vi "Main.vi"() -> ()   [LabVIEW 2018, in "Popup.lvlib"]
doc: "This template is based from the Queued Message Handler design pattern and the Queued Message Handler Project Template that ships with LabVIEW 2014.\n\nThe main difference is that the Queue is private to this module and communication between modules is done via Broadcast and Requests events.\n\nRequests events are wrapped via public API methods and are handled in the Event handler loop in this VI.\nAny module can register for Broadcast events sent by this module.\n\nThe Event Handling Loop generates messages based on user interface actions.\n\nThe Message Handling Loop processes messages generated by the Event Handling Loop, or by other messages. The messages are string values, so new messages can be added easily to the Message Cases case structure in the Message Handling Loop. Each message cluster can also provide an optional value for Message Data, which is a variant that can be converted to whatever message-specific data is required.\n_____\nBased on Delacor QMH Project Template 3.1.0.34."
uses:
  Popup.lvlib
  <vilib>/Delacor/Delacor QMH/Libraries/Cloneable Module Admin_class/Delacor_lib_QMH_Cloneable Module Admin.lvclass
  C:/Program Files (x86)/National Instruments/LabVIEW 2018/vi.lib/Delacor/Delacor QMH/Libraries/Module Admin_class/Delacor_lib_QMH_Module Admin.lvclass
  <vilib>/MGI/Panel Manager/Panel/Panel/Panel.lvclass
  <vilib>/Utility/miscctls.llb/LVPointTypeDef.ctl
  Module Data--cluster.ctl
  <vilib>/Delacor/Delacor QMH/Libraries/Message Queue_class/Delacor_lib_QMH_Message Queue.lvclass/Delacor_lib_QMH_Message Queue.ctl
  <vilib>/Delacor/Delacor QMH/Libraries/Cloneable Module Admin_class/Delacor_lib_QMH_Cloneable Module Admin.lvclass/Delacor_lib_QMH_Cloneable Module Admin.ctl
  Stop Argument--cluster.ctl
  <vilib>/Delacor/Delacor QMH/Libraries/Module Admin_class/Delacor_lib_QMH_Module Admin.lvclass/Delacor_lib_QMH_Module Admin.ctl
  modify panl  origin position Argument--cluster.ctl
  Modify window front Argument--cluster.ctl
  Modify Title name Argument--cluster.ctl
  <vilib>/Utility/miscctls.llb/LVRectTypeDef.ctl
  <vilib>/Delacor/Delacor QMH/Libraries/Message Queue_class/Delacor_lib_QMH_Enqueue Message (Single).vi
  <vilib>/Delacor/Delacor QMH/Libraries/Cloneable Module Admin_class/Delacor_lib_QMH_Get Module ID.vi
  <vilib>/Delacor/Delacor QMH/Libraries/Module Admin_class/Delacor_lib_QMH_Get External Launch.vi
  <vilib>/Utility/error.llb/Error Cluster From Error Code.vi
  <vilib>/ErrorRing/Error Ring.xnode
  <vilib>/Delacor/Delacor QMH/Libraries/Message Queue_class/Delacor_lib_QMH_Message Queue.lvclass
  Clone Registration/Clone Registration.lvlib
  <vilib>/MGI/Panel Manager/Panel/Panel Helper/Panel Helper.lvclass
panel:
  in  "显示字符串":string
  in  "Panel":refnum<class "Panel.lvclass">
  in  "Simulate MHL Error":bool
  in  "Simulate EHL Error":bool
  out "error out":errorcluster
  in  "Module Admin":refnum<class "Delacor_lib_QMH_Cloneable Module Admin.lvclass">
  out "Status":string
  # "一个模块涵盖所有弹窗\n所有对应操作全部通过命令下发"
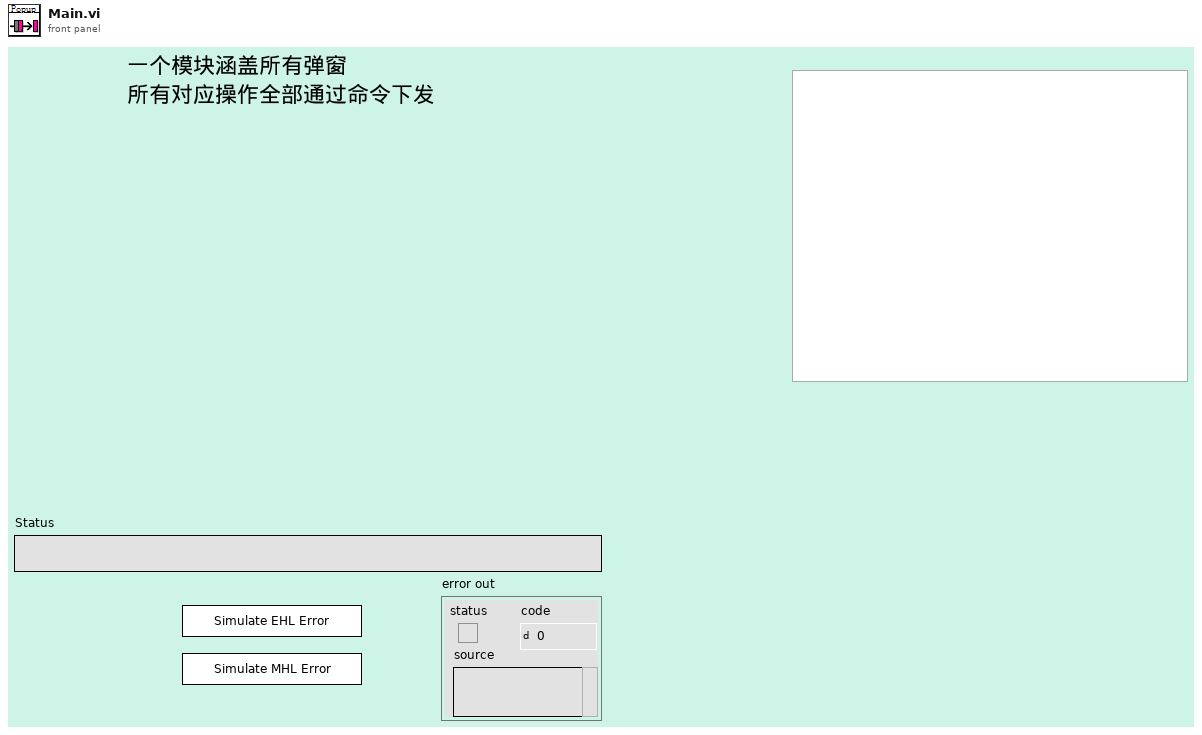
[diagram p1: front panel]
types:
  T1 = typedef "LVPointTypeDef.ctl" = cluster{"Horizontal":i16, "Vertical":i16}
  T2 = typedef "Popup.lvlib/Request Events--cluster.ctl" = cluster{"Stop Module":refnum<user-event>, "Show Panel":refnum<user-event>, "Hide Panel":refnum<user-event>, "Show Diagram":refnum<user-event>, "Get Module Execution Status":refnum<user-event>, "Change Panel":refnum<user-event>, "modify panl  origin position":refnum<user-event>, "Modify window front":refnum<user-event>, "Modify Title name":refnum<user-event>}
  T3 = typedef "Panel.lvlib/Panel Helper.lvclass/Panel Events.ctl" = cluster{"My Panel":refnum<user-event>, "Top Level Initialized":refnum<user-event>}
  T4 = typedef "Popup.lvlib/Module Data--cluster.ctl" = cluster{"Status":string, "本VI":refnum<vi>}
  T5 = typedef "Popup.lvlib/Stop Argument--cluster.ctl" = cluster{"Origin":string, "Module ID":i32, "Exit via Stop Module Req?":bool, "Wait for Module to stop?":bool}
  T6 = typedef "Popup.lvlib/modify panl  origin position Argument--cluster.ctl" = cluster{"Module ID":i32, "Origin":cluster{"Horizontal":i16, "Vertical":i16}}
  T7 = typedef "Popup.lvlib/Modify window front Argument--cluster.ctl" = cluster{"Module ID":i32, "Bottom":i16, "Right":i16, "Top":i16, "Left":i16}
  T8 = typedef "Popup.lvlib/Modify Title name Argument--cluster.ctl" = cluster{"Module ID":i32, "标题":string}
  T9 = enum32{"invalid lock state", "Not Locked", "Locked (No Password)", "Password-protected"}
  T10 = typedef "LVRectTypeDef.ctl" = cluster{"Left":i16, "Top":i16, "Right":i16, "Bottom":i16}
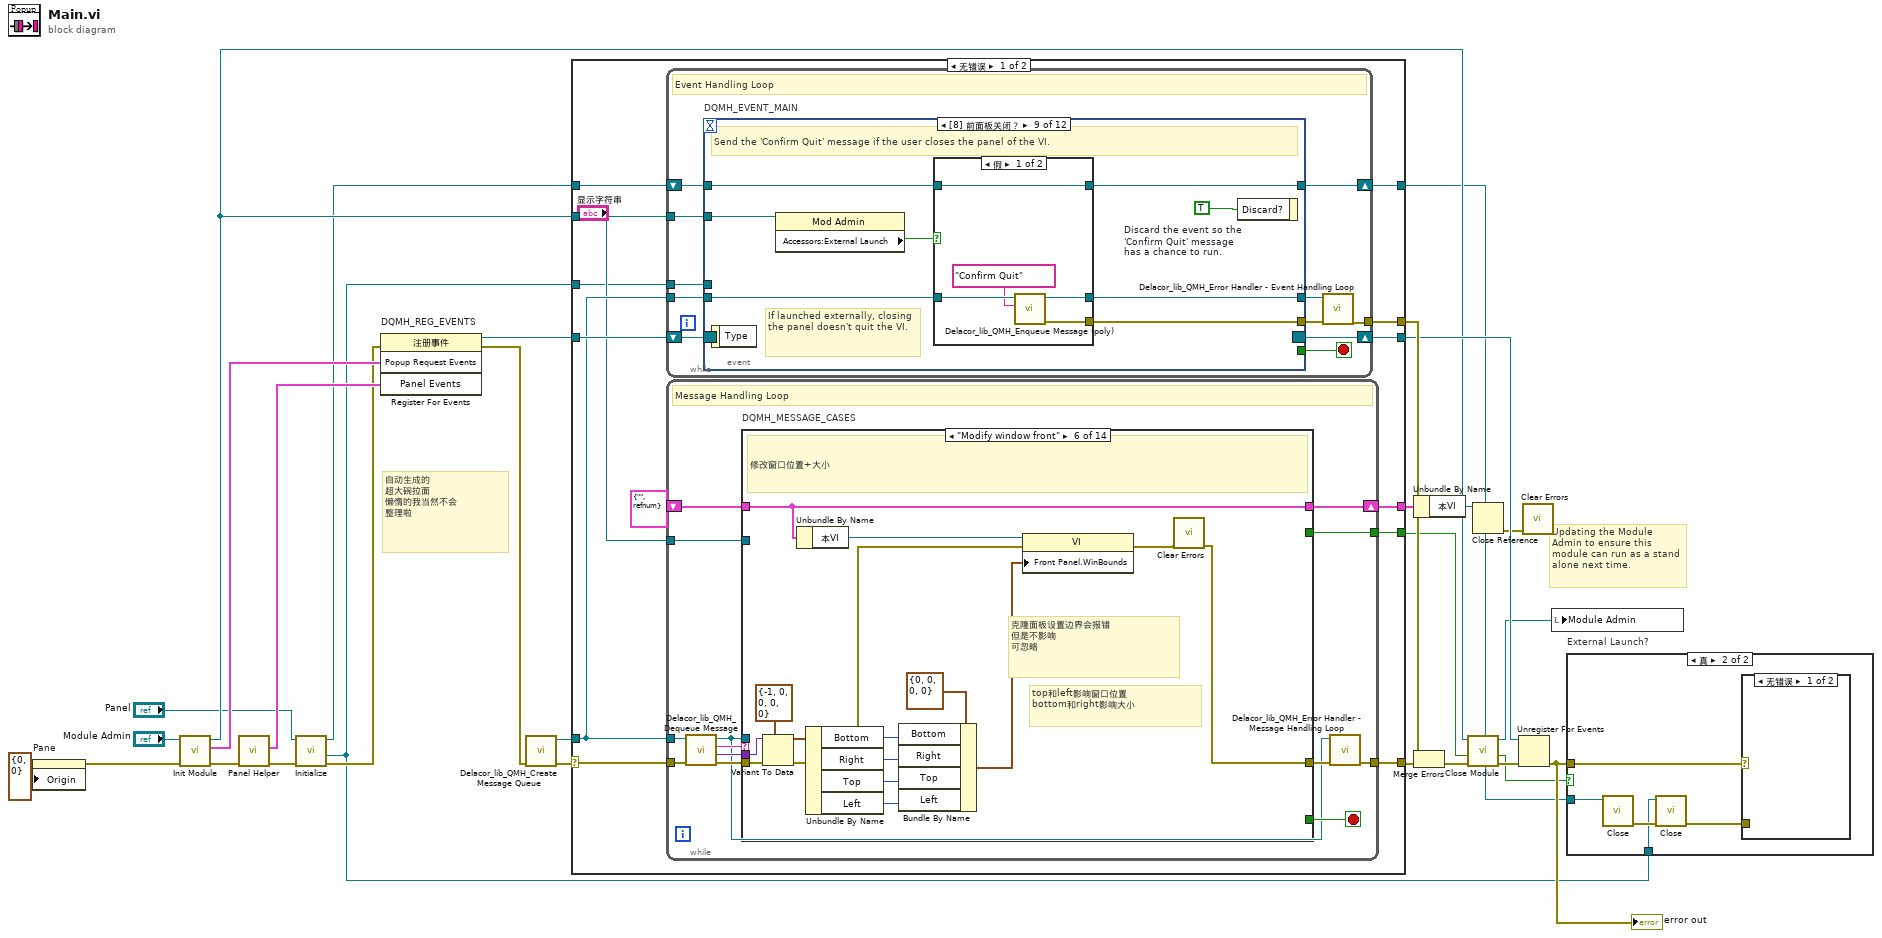
[diagram p0: block diagram]
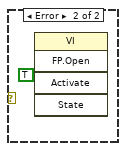
[diagram p3: hidden frame]
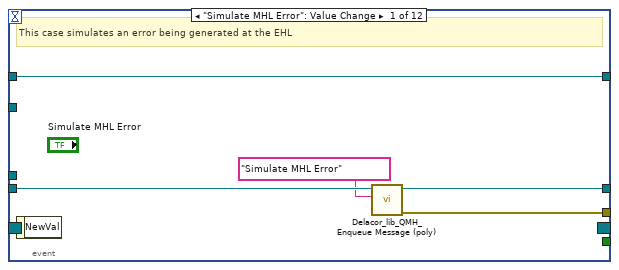
[diagram p4: hidden frame]
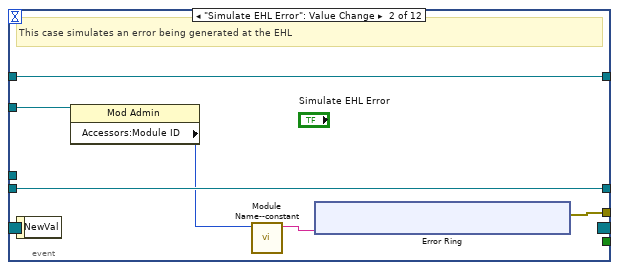
[diagram p5: hidden frame]
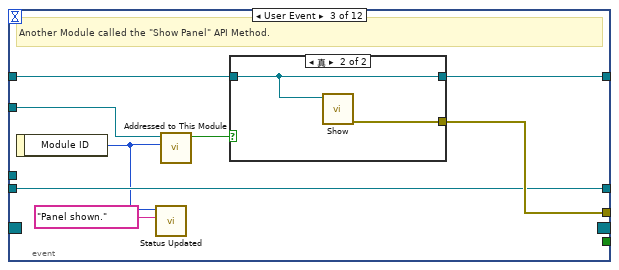
[diagram p6: hidden frame]
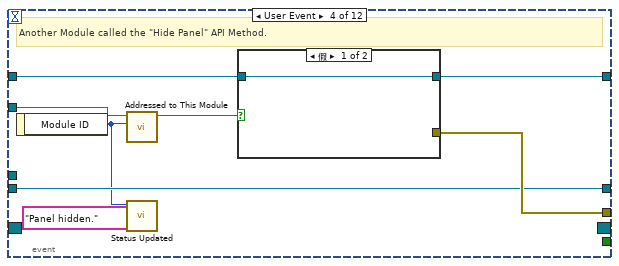
[diagram p8: hidden frame]
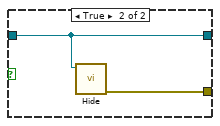
[diagram p9: hidden frame]
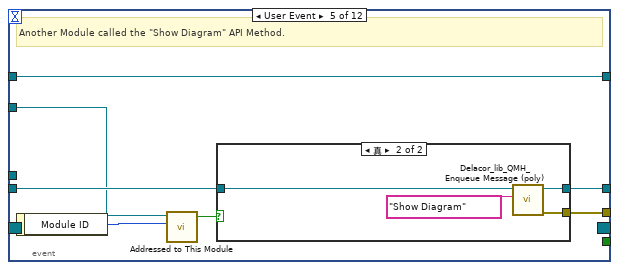
[diagram p10: hidden frame]
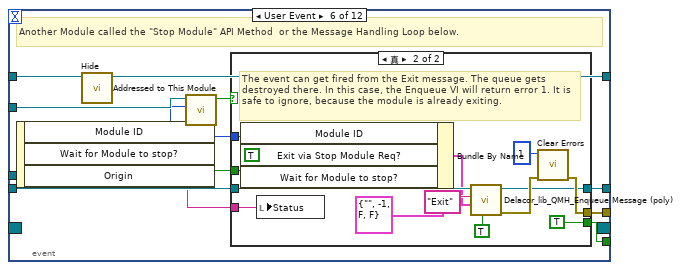
[diagram p12: hidden frame]
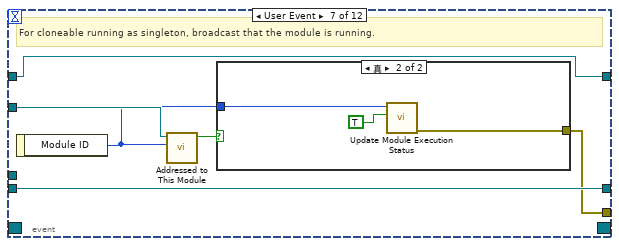
[diagram p14: hidden frame]
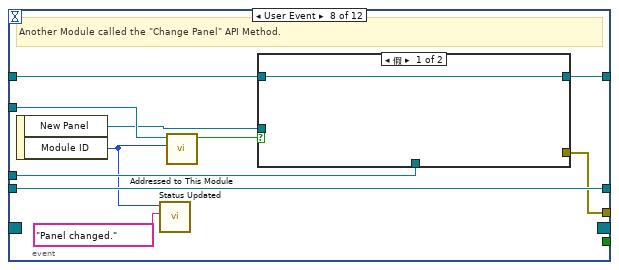
[diagram p16: hidden frame]
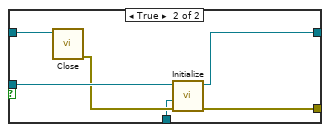
[diagram p17: hidden frame]
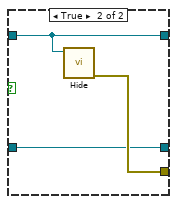
[diagram p18: hidden frame]
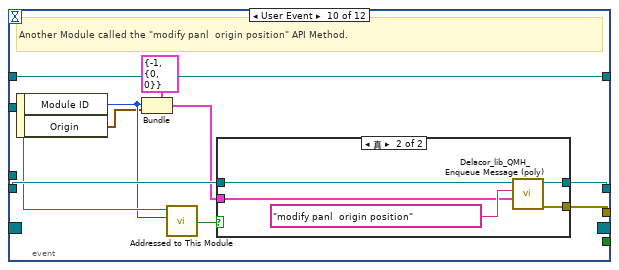
[diagram p19: hidden frame]
diagram:
  # "自动生成的\n超大碗拉面\n懒惰的我当然不会\n整理啦"
  # "Updating the Module Admin to ensure this module can run as a stand alone next time."
  n1 = property on="Pane" class="Pane"("Origin"=T1 {"Horizontal"=0, "Vertical"=0}) -> (error out=w4:errorcluster)  [unwired: 2 in, 1 out]
  n2 = call "Init Module.vi"("error in (no error)"=w4, "Cloneable Module Admin in"="Module Admin") -> ("error out"=w14:errorcluster, "Popup Request Events"=w24:T2, "Cloneable Module Admin out"=w20:refnum<class "Delacor_lib_QMH_Cloneable Module Admin.lvclass">)  [unwired: 7 in]
  n3 = call <vilib>:"Panel Helper.vi"("Error In"=w14) -> ("Error Out"=w10:errorcluster, "Panel Events"=w13:T3)  [unwired: 8 in, 1 out]
  n4 = call <vilib>:"Initialize.vi"("error in (no error)"=w10, "Panel In"="Panel") -> ("error out"=w9:errorcluster, "My Helper out"=w6:refnum<class "Panel Helper.lvclass">, "Panel Out"=w7:refnum<class "Panel.lvclass">)  [unwired: 7 in]
  n5 = register-events "DQMH_REG_EVENTS"(error in=w9, w24, w13) -> (reference out=w25:refnum<event-registration>, error out=w11:errorcluster)  [unwired: 1 in]
  n6 = call <vilib>:"Delacor_lib_QMH_Create Message Queue.vi"("error in"=w11) -> ("error out"=w15:errorcluster, "Message Queue"=w23:refnum<class "Delacor_lib_QMH_Message Queue.lvclass">)  [unwired: 9 in]
  n7 = case shown="无错误" w15 {
    selector: w15 -> [w36 w403]
    tunnel: [w42 w403] -> w27
    tunnel: [w41 w404] -> w26
    tunnel: w25 -> [w39 w404]
    tunnel: w23 -> [w38 _]
    tunnel: [w37 _] -> w28
    tunnel: w20 -> [w35 w399]
    tunnel: [w34 _] -> w18
    tunnel: w6 -> [w31 _]
    tunnel: w7 -> [w33 w396]
    tunnel: [w32 w396] -> w12
    tunnel: [w30 _] -> w3
    frame No Error {
      n8 = while {
        tunnel: w38 -> [w53]
        shift-right: [w51] -> w41
        shift-left: w39 -> [w52]
        tunnel: [w47] -> w37
        tunnel: w35 -> [w46]
        shift-right: [w44] -> w32
        shift-left: w33 -> [w45]
        tunnel: w31 -> [w43]
        stop <- w49 stop-if-true
        # "Event Handling Loop"
        n9 = event "DQMH_EVENT_MAIN" shown="[8] 前面板关闭？" {
          selector: w52 -> [_ _ _ _ _ _ _ _ _ _ _ _]
          dyn-events: [_ _ _ _ _ _ _ _ _ _ _ _] -> w51
          timeout: _ -> [_ _ _ _ _ _ _ _ _ _ _ _]
          tunnel: [_ _ _ _ _ w110 _ _ _ _ _ _] -> w49
          tunnel: w53 -> [w58 w64 w74 w85 w100 w113 w134 w146 w158 w181 w200 w216]
          tunnel: [w56 w63 w79 w90 w96 w115 w133 w144 w157 w173 w189 w208] -> w50
          tunnel: [w57 w64 w74 w85 w99 w114 w134 w146 w159 w180 w199 w215] -> w48
          tunnel: w46 -> [_ w62 w77 w88 w97 w112 w135 w149 w163 w178 w197 w213]
          tunnel: w45 -> [w54 w59 w76 w86 w94 w106 w131 w148 w162 w182 w201 w217]
          tunnel: [w54 w59 w75 w87 w94 w106 w131 w147 w161 w182 w201 w217] -> w44
          tunnel: w43 -> [_ _ _ _ _ _ _ w143 _ _ _ _]
          event "Simulate MHL Error": Value Change {
            # "This case simulates an error being generated at the EHL"
            n10 = event-data() -> ()  [unwired: 1 in, 1 out]
            n11 = call-poly <vilib>:"Delacor_lib_QMH_Enqueue Message (poly).vi"("Message"="Simulate MHL Error", "Message Queue in"=w58) -> ("error out"=w56:errorcluster, "Message Queue out"=w57:refnum<class "Delacor_lib_QMH_Message Queue.lvclass">)  [unwired: 8 in]
          }
          event "Simulate EHL Error": Value Change {
            # "This case simulates an error being generated at the EHL"
            n12 = event-data() -> ()  [unwired: 1 in, 1 out]
            n13 = property class="Mod Admin"(reference=w62) -> ("Accessors:Module ID"=w61:i32)  [unwired: 1 in, 2 out]
            n14 = call "Module Name--constant.vi"("Module ID"=w61) -> ("Module Name"=w60:string)  [unwired: 10 in]
            n15 = xnode "Error Ring"("参数 0"=w60) -> ("错误输出"=w63:errorcluster)
          }
          event User Event {
            # "Another Module called the \"Show Panel\" API Method."
            n16 = event-data() -> ("Module ID"=w72:i32)  [unwired: 1 in]
            n17 = call "Status Updated.vi"("Status"="Panel shown." ("format string"), "Module ID"=w72) -> ()  [unwired: 9 in, 1 out]
            n18 = call "Addressed to This Module.vi"("Module ID from Argument"=w72, "Module Admin"=w77) -> ("Addressed to this instance?"=w78:bool)  [unwired: 8 in, 1 out]
            n19 = case shown="真" w78 {
              tunnel: [_ w81] -> w79
              tunnel: w76 -> [w80 w82]
              tunnel: [w80 w82] -> w75
              frame False {
              }
              frame True {
                n20 = call <vilib>:"Show.vi"("Panel in"=w82) -> ("Error Out"=w81:errorcluster)  [unwired: 10 in]
              }
            }
          }
          event User Event {
            # "Another Module called the \"Hide Panel\" API Method."
            n21 = event-data() -> ("Module ID"=w83:i32)  [unwired: 1 in]
            n22 = call "Addressed to This Module.vi"("Module ID from Argument"=w83, "Module Admin"=w88) -> ("Addressed to this instance?"=w89:bool)  [unwired: 8 in, 1 out]
            n23 = call "Status Updated.vi"("Status"="Panel hidden." ("format string"), "Module ID"=w83) -> ()  [unwired: 9 in, 1 out]
            n24 = case shown="假" w89 {
              tunnel: [_ w92] -> w90
              tunnel: [w91 w93] -> w87
              tunnel: w86 -> [w91 w93]
              frame False {
              }
              frame True {
                n25 = call <vilib>:"Hide.vi"("Panel In"=w93) -> ("Error Out"=w92:errorcluster)  [unwired: 10 in]
              }
            }
          }
          event User Event {
            # "Another Module called the \"Show Diagram\" API Method."
            n26 = event-data() -> ("Module ID"=w95:i32)  [unwired: 1 in]
            n27 = call "Addressed to This Module.vi"("Module ID from Argument"=w95, "Module Admin"=w97) -> ("Addressed to this instance?"=w98:bool)  [unwired: 8 in, 1 out]
            n28 = case shown="真" w98 {
              tunnel: w100 -> [w101 w105]
              tunnel: [w101 w104] -> w99
              tunnel: [_ w102] -> w96
              frame False {
              }
              frame True {
                n29 = call-poly <vilib>:"Delacor_lib_QMH_Enqueue Message (poly).vi"("Message"="Show Diagram", "Message Queue in"=w105) -> ("error out"=w102:errorcluster, "Message Queue out"=w104:refnum<class "Delacor_lib_QMH_Message Queue.lvclass">)  [unwired: 8 in]
              }
            }
          }
          event User Event {
            # "Another Module called the \"Stop Module\" API Method  or the Message Handling Loop below."
            n30 = event-data() -> ("Module ID"=w108:i32, "Wait for Module to stop?"=w109:bool, "Origin"=w107:string)  [unwired: 1 in]
            n31 = call <vilib>:"Hide.vi"("Panel In"=w106) -> ()  [unwired: 10 in, 1 out]
            n32 = call "Addressed to This Module.vi"("Module ID from Argument"=w108, "Module Admin"=w112) -> ("Addressed to this instance?"=w111:bool)  [unwired: 8 in, 1 out]
            n33 = case shown="真" w111 {
              tunnel: [_ w126] -> w115
              tunnel: [w116 w125] -> w114
              tunnel: w113 -> [w116 w124]
              tunnel: [_ TRUE] -> w110
              tunnel: w109 -> [_ w119]
              tunnel: w108 -> [_ w121]
              tunnel: w107 -> [_ w117]
              frame False {
              }
              frame True {
                # "The event can get fired from the Exit message. The queue gets destroyed there. In this case, the Enqueue VI will return error 1. It is safe to ignore, because the module is already exiting."
                n34 = Bundle By Name(cluster=T5 {"Origin"="", "Module ID"=-1, "Exit via Stop Module Req?"=FALSE, "Wait for Module to stop?"=FALSE} ("Stop Argument"), "Module ID"=w121, "Exit via Stop Module Req?"=TRUE, "Wait for Module to stop?"=w119) -> (w118:T5)
                n35 = local write "Status"(w117) -> ()
                n36 = call-poly <vilib>:"Delacor_lib_QMH_Enqueue Message (poly).vi"("Priority Message? (F)"=TRUE, "Message Data"=w118, "Message"="Exit", "Message Queue in"=w124) -> ("error out"=w129:errorcluster, "Message Queue out"=w125:refnum<class "Delacor_lib_QMH_Message Queue.lvclass">)  [unwired: 6 in]
                n37 = call <vilib>:"Clear Errors.vi"("error in (no error)"=w129, "specific error code to clear (0: all)"=1) -> ("error out"=w126:errorcluster)  [unwired: 4 in, 1 out]
              }
            }
          }
          event User Event {
            # "For cloneable running as singleton, broadcast that the module is running."
            n38 = event-data() -> ("Module ID"=w132:i32)  [unwired: 1 in]
            n39 = call "Addressed to This Module.vi"("Module ID from Argument"=w132, "Module Admin"=w135) -> ("Addressed to this instance?"=w136:bool)  [unwired: 8 in, 1 out]
            n40 = case shown="真" w136 {
              tunnel: [_ w139] -> w133
              tunnel: w132 -> [_ w138]
              frame False {
              }
              frame True {
                n41 = call "Update Module Execution Status.vi"("Running?"=TRUE, "Module ID"=w138) -> ("error out"=w139:errorcluster)  [unwired: 9 in]
              }
            }
          }
          event User Event {
            # "Another Module called the \"Change Panel\" API Method."
            n42 = event-data() -> ("New Panel"=w145:refnum<class "Panel.lvclass">, "Module ID"=w141:i32)  [unwired: 1 in]
            n43 = call "Status Updated.vi"("Status"="Panel changed.", "Module ID"=w141) -> ()  [unwired: 9 in, 1 out]
            n44 = call "Addressed to This Module.vi"("Module ID from Argument"=w141, "Module Admin"=w149) -> ("Addressed to this instance?"=w140:bool)  [unwired: 8 in, 1 out]
            n45 = case shown="假" w140 {
              tunnel: w148 -> [w150 w156]
              tunnel: [w150 w154] -> w147
              tunnel: w145 -> [_ w155]
              tunnel: [_ w152] -> w144
              tunnel: w143 -> [_ w151]
              frame False {
              }
              frame True {
                n46 = call-dynamic <vilib>:"Close.vi"("Panel In"=w156) -> ("Error Out"=w153:errorcluster)  [unwired: 10 in]
                n47 = call <vilib>:"Initialize.vi"("error in (no error)"=w153, "My Helper in"=w151, "Panel In"=w155) -> ("error out"=w152:errorcluster, "Panel Out"=w154:refnum<class "Panel.lvclass">)  [unwired: 6 in, 1 out]
              }
            }
          }
          event Panel Close? {
            w164 = TRUE  # Discard the event so the 'Confirm Quit' message has a chance to run.
            # "If launched externally, closing the panel doesn't quit the VI."
            # "Send the 'Confirm Quit' message if the user closes the panel of the VI."
            n48 = event-data() -> ()  [unwired: 1 in, 1 out]
            n49 = property class="Mod Admin"(reference=w163) -> ("Accessors:External Launch"=w160:bool)  [unwired: 1 in, 2 out]
            n50 = case "条件结构" shown="假" w160 {
              tunnel: w162 -> [w167 w172]
              tunnel: [w167 w172] -> w161
              tunnel: [w166 w171] -> w157
              tunnel: [w168 w170] -> w159
              tunnel: w158 -> [w169 w170]
              frame False {
                n51 = call-poly <vilib>:"Delacor_lib_QMH_Enqueue Message (poly).vi"("Message"="Confirm Quit", "Message Queue in"=w169) -> ("error out"=w166:errorcluster, "Message Queue out"=w168:refnum<class "Delacor_lib_QMH_Message Queue.lvclass">)  [unwired: 8 in]
              }
              frame True {
                n52 = call <vilib>:"Hide.vi"("Panel In"=w172) -> ("Error Out"=w171:errorcluster)  [unwired: 10 in]
              }
            }
            n53 = event-data("Discard?"=w164) -> ()  [unwired: 1 in, 1 out]
          }
          event User Event {
            # "Another Module called the \"modify panl  origin position\" API Method."
            n54 = event-data() -> ("Module ID"=w175:i32, "Origin"=w174:cluster{"Horizontal":i16, "Vertical":i16})  [unwired: 1 in]
            n55 = Bundle(cluster=T6 {"Module ID"=-1, "Origin"={"Horizontal"=0, "Vertical"=0}} ("modify panl  origin position Argument"), "Module ID"=w175, "Origin"=w174) -> (w176:T6)
            n56 = call "Addressed to This Module.vi"("Module ID from Argument"=w175, "Module Admin"=w178) -> ("Addressed to this instance?"=w179:bool)  [unwired: 8 in, 1 out]
            n57 = case "条件结构" shown="真" w179 {
              tunnel: w181 -> [w183 w188]
              tunnel: [w183 w187] -> w180
              tunnel: w176 -> [_ w185]
              tunnel: [_ w184] -> w173
              frame False {
              }
              frame True {
                n58 = call-poly <vilib>:"Delacor_lib_QMH_Enqueue Message (poly).vi"("Message Data"=w185, "Message"="modify panl  origin position", "Message Queue in"=w188) -> ("error out"=w184:errorcluster, "Message Queue out"=w187:refnum<class "Delacor_lib_QMH_Message Queue.lvclass">)  [unwired: 7 in]
              }
            }
          }
          event User Event {
            # "Another Module called the \"Modify window front\" API Method."
            n59 = event-data() -> ("Module ID"=w194:i32, "Bottom"=w193:i16, "Right"=w192:i16, "Top"=w191:i16, "Left"=w190:i16)  [unwired: 1 in]
            n60 = Bundle(cluster=T7 {"Module ID"=-1, "Bottom"=0, "Right"=0, "Top"=0, "Left"=0} ("Modify window front Argument"), "Module ID"=w194, "Bottom"=w193, "Right"=w192, "Top"=w191, "Left"=w190) -> (w195:T7)
            n61 = call "Addressed to This Module.vi"("Module ID from Argument"=w194, "Module Admin"=w197) -> ("Addressed to this instance?"=w198:bool)  [unwired: 8 in, 1 out]
            n62 = case "条件结构" shown="真" w198 {
              tunnel: w200 -> [w202 w207]
              tunnel: [w202 w206] -> w199
              tunnel: w195 -> [_ w204]
              tunnel: [_ w203] -> w189
              frame False {
              }
              frame True {
                n63 = call-poly <vilib>:"Delacor_lib_QMH_Enqueue Message (poly).vi"("Message Data"=w204, "Message"="Modify window front", "Message Queue in"=w207) -> ("error out"=w203:errorcluster, "Message Queue out"=w206:refnum<class "Delacor_lib_QMH_Message Queue.lvclass">)  [unwired: 7 in]
              }
            }
          }
          event User Event {
            # "Another Module called the \"Modify Title name\" API Method."
            n64 = event-data() -> ("Module ID"=w210:i32, "标题"=w209:string)  [unwired: 1 in]
            n65 = Bundle(cluster=T8 {"Module ID"=-1, "标题"=""} ("Modify Title name Argument"), "Module ID"=w210, "标题"=w209) -> (w211:T8)
            n66 = call "Addressed to This Module.vi"("Module ID from Argument"=w210, "Module Admin"=w213) -> ("Addressed to this instance?"=w214:bool)  [unwired: 8 in, 1 out]
            n67 = case "条件结构" shown="真" w214 {
              tunnel: w216 -> [w218 w223]
              tunnel: [w218 w222] -> w215
              tunnel: w211 -> [_ w220]
              tunnel: [_ w219] -> w208
              frame False {
              }
              frame True {
                n68 = call-poly <vilib>:"Delacor_lib_QMH_Enqueue Message (poly).vi"("Message Data"=w220, "Message"="Modify Title name", "Message Queue in"=w223) -> ("error out"=w219:errorcluster, "Message Queue out"=w222:refnum<class "Delacor_lib_QMH_Message Queue.lvclass">)  [unwired: 7 in]
              }
            }
          }
        }
        n69 = call-dynamic "Delacor_lib_QMH_Error Handler - Event Handling Loop.vi"("error in"=w50, "Message Queue in"=w48) -> ("dup error in"=w47:errorcluster)  [unwired: 8 in, 1 out]
      }
      n70 = while {
        tunnel: w38 -> [w228]
        shift-right: [w234] -> w30
        shift-left: T4 {"Status"="", "本VI"=refnum} ("Data Cluster") -> [w235]
        tunnel: w36 -> [w232]
        tunnel: [w226] -> w42
        tunnel: w35 -> [w225]
        tunnel: [w224] -> w34
        stop <- w233 stop-if-true
        # "Message Handling Loop"
        n71 = call-dynamic "Delacor_lib_QMH_Dequeue Message.vi"("error in"=w232, "Message Queue in"=w228) -> ("error out"=w231:errorcluster, "Message Data"=w229:variant, "Message"=w230:string, "Message Queue out"=w227:refnum<class "Delacor_lib_QMH_Message Queue.lvclass">)  [unwired: 6 in]
        n72 = case "DQMH_MESSAGE_CASES" shown="\"Modify window front\"" w230 {
          selector: w230 -> [_ _ _ _ _ _ _ _ _ _ _ _ _ w385]
          tunnel: w227 -> [_ _ _ _ _ _ _ _ _ w330 _ w363 w379 _]
          tunnel: w231 -> [w248 w256 w261 w282 w298 w313 w322 w325 w328 w339 w352 w362 w381 _]
          tunnel: [w243 w257 w260 w280 w292 w300 w314 w323 w326 w329 w350 w361 w375 w386] -> w236
          tunnel: w235 -> [w247 w258 w262 w281 w297 w310 w318 w324 w327 w338 w351 w366 w378 w387]
          tunnel: [w246 w258 w262 w281 w297 w310 w318 w324 w327 w338 w351 w366 w378 w387] -> w234
          tunnel: [_ _ _ _ _ _ _ _ _ _ _ _ w377 _] -> w233
          tunnel: w229 -> [_ w255 _ _ w296 w312 w321 _ _ w337 _ _ w371 _]
          tunnel: w225 -> [w241 w250 w259 _ _ _ _ _ _ w334 w347 _ w367 w383]
          tunnel: [_ _ _ _ _ _ _ _ _ _ _ _ w369 _] -> w224
          frame "Initialize" {
            w245 = "Initial Message" ("Initial Message")
            # "#CodeNeeded - Initialize the appearance of the front panel."
            # "#CodeNeeded - Initialize your state data here."
            # "Initialize - Any operation that needs to be done before the module can receive messages. Synchronize Caller Events.vi will inform Start Module.vi that the module has launched and is ready to receive messages. Module Did Init.vi will broadcast that the module initialized."
            n73 = call "Synchronize Caller Events.vi"("error in (no error)"=w248, "Module Admin"=w241) -> ("error out"=w239:errorcluster, "Module Admin out"=w240:refnum<class "Delacor_lib_QMH_Cloneable Module Admin.lvclass">)  [unwired: 8 in]
            n74 = property class="Mod Admin"(reference=w240) -> ("Accessors:Module ID"=w242:i32)  [unwired: 1 in, 2 out]
            n75 = call "Module Name--constant.vi"("Module ID"=w242) -> ("Module Name"=w238:string)  [unwired: 10 in]
            n76 = control-ref of="本VI"() -> (w237:refnum<vi>)
            n77 = Bundle By Name(cluster=w247, "Status"=w245, "本VI"=w237) -> (w246:T4)
            n78 = local write "Status"(w245) -> ()
            n79 = call "Module Did Init.vi"("error in (no error)"=w239, "Initialized?"=TRUE, "Origin"=w238, "Module ID"=w242) -> ("error out"=w243:errorcluster)  [unwired: 7 in]
          }
          frame "Update Display" {
            # "Broadcast updated status to any VI registered to listen to this module's broadcast events."
            # "Convert the message data to a string to display in the Status indicator."
            # "#CodeRecommended - If you wish to decouple the Message Handling Loop from your user interface, consider creating User Events (like the \"Stop\" event in this VI) to message the Event Handling Loop whenever the user interface needs updating."
            # "Update Display - Update user interface here."
            n80 = Variant To Data(error in=w256, type="" ("空字符串常量"), Variant=w255) -> (data=w253:string, error out=w252:errorcluster)
            "Status" <- w253
            n81 = property class="Mod Admin"(reference=w250) -> ("Accessors:Module ID"=w249:i32)  [unwired: 1 in, 2 out]
            n82 = call "Status Updated.vi"("error in (no error)"=w252, "Status"=w253, "Module ID"=w249) -> ("error out"=w251:errorcluster)  [unwired: 8 in]
            n83 = Merge Errors(w251) -> (w257:errorcluster)
          }
          frame "Show Diagram" {
            # "Show Diagram - Show the block diagram of this VI. Used as a debugging tool. There is a button in the module tester that fires the Show Diagram request, which runs this message. Note that the diagram will not be displayed if it is password-protected and the password is not in the cache."
            n84 = disable-structure shown="RUN_TIME_ENGINE==False" {
              disable-tunnel: [w271 w279] -> w260
              disable-tunnel: w261 -> [w270 w279]
              disable-tunnel: w259 -> [w263 _]
              frame condition #0 (active) {
                # "functionality not available in exe"
                n85 = invoke class="VI" method="Lock State.Get"(error in=w270) -> (error out=w269:errorcluster, "Get Lock State"=w268:T9, "pwd in cache"=w265:bool)  [unwired: 3 in, 1 out]
                n86 = Equal?(x=T9."Password-protected", y=w268) -> (x = y?=w266:bool)
                n87 = Compound Arithmetic op=AND(w266, invert w265) -> (w264:bool)
                n88 = case shown="假" w264 {
                  tunnel: [w276 w278] -> w271
                  tunnel: w269 -> [w275 w278]
                  tunnel: w263 -> [w272 _]
                  frame False {
                    n89 = property class="Mod Admin"(reference=w272) -> ("Accessors:Module ID"=w273:i32)  [unwired: 1 in, 2 out]
                    n90 = property class="VI"(error in=w275, "BDWin.Open"=TRUE ("Block Diagram Window:Open")) -> (error out=w276:errorcluster)  [unwired: 1 in, 1 out]
                    n91 = call "Status Updated.vi"("Status"="Block Diagram shown." ("format string"), "Module ID"=w273) -> ()  [unwired: 9 in, 1 out]
                  }
                  frame True {
                    # "Password-protected VI, and the password is not in the cache. Do not show the diagram."
                  }
                }
              }
              frame condition #1 {
              }
            }
          }
          frame "--- Module Specific ---" {
            # "Separator -- The following cases handle messages specific to this Module."
            n92 = Merge Errors(w282) -> (w280:errorcluster)
          }
          frame "modify panl  origin position" {
            # "修改前面板原点位位置以达到换一块新的地方出来"
            n93 = Variant To Data(error in=w298, type=T6 {"Module ID"=-1, "Origin"={"Horizontal"=0, "Vertical"=0}} ("modify panl  origin position Argument"), Variant=w296) -> (data=w294:T6, error out=w293:errorcluster)
            n94 = Unbundle By Name(w294) -> ("Module ID"=w289:i32, "Origin"=w291:cluster{"Horizontal":i16, "Vertical":i16})
            n95 = Unbundle By Name(w291) -> ("Horizontal"=w287:i16, "Vertical"=w283:i16)
            n96 = property on="Pane" class="Pane"(error in=w293, "Origin"=w291) -> (error out=w288:errorcluster)  [unwired: 1 in, 1 out]
            n97 = Format Into String(format string="（%d，%d）" ("格式字符串"), initial string="modified origin position" ("输入字符串"), error in=w288, w287, w283) -> (resulting string=w286:string, error out=w285:errorcluster)
            n98 = call "Status Updated.vi"("error in (no error)"=w285, "Status"=w286, "Module ID"=w289) -> ("error out"=w292:errorcluster)  [unwired: 8 in]
          }
          frame "Modify window front" {
            # "top和left影响窗口位置\nbottom和right影响大小"
            # "克隆面板设置边界会报错\n但是不影响\n可忽略"
            # "修改窗口位置+大小"
            n99 = Variant To Data(error in=w313, type=T7 {"Module ID"=-1, "Bottom"=0, "Right"=0, "Top"=0, "Left"=0} ("Modify window front Argument"), Variant=w312) -> (data=w306:T7, error out=w308:errorcluster)
            n100 = Unbundle By Name(w310) -> ("本VI"=w309:refnum<vi>)
            n101 = Unbundle By Name(w306) -> ("Bottom"=w305:i16, "Right"=w304:i16, "Top"=w303:i16, "Left"=w302:i16)
            n102 = Bundle By Name(cluster=T10 {"Left"=0, "Top"=0, "Right"=0, "Bottom"=0} ("前面板窗口:窗口边界"), "Bottom"=w305, "Right"=w304, "Top"=w303, "Left"=w302) -> (w299:T10)
            n103 = property class="VI"(reference=w309, error in=w308, "Front Panel.WinBounds"=w299) -> (error out=w301:errorcluster)  [unwired: 1 out]
            n104 = call <vilib>:"Clear Errors.vi"("error in (no error)"=w301) -> ("error out"=w300:errorcluster)  [unwired: 5 in, 1 out]
          }
          frame "Modify Title name" {
            # "修改标题栏"
            n105 = Variant To Data(error in=w322, type=T8 {"Module ID"=-1, "标题"=""} ("Modify Title name Argument"), Variant=w321) -> (data=w319:T8, error out=w315:errorcluster)
            n106 = Unbundle By Name(w319) -> ("标题"=w316:string)
            n107 = Unbundle By Name(w318) -> ("本VI"=w317:refnum<vi>)
            n108 = property class="VI"(reference=w317, error in=w315, "Front Panel.Title"=w316) -> (error out=w314:errorcluster)  [unwired: 1 out]
          }
          frame "---Copy This Frame---" {
            # "Duplicate this frame when creating new messages.  Change this comment in the duplicated frame to describe this message."
            n109 = Merge Errors(w325) -> (w323:errorcluster)
          }
          frame "--- Exit and Error Handling---" {
            # "Separator - the following cases handle errors and exit messages."
            n110 = Merge Errors(w328) -> (w326:errorcluster)
          }
          frame "Error" {
            # "#CodeRecommended - If you ever change the name of this \"Error\" message, you'll need to update the name in the Check Loop Error.vi as well."
            # "#CodeRecommended - If the module is running in standalone mode (External Launch = FALSE), this code will pop up an error dialog and call the 'Exit' message if an error occurs. Add more fine-grained error handling here."
            # "Error - Check the error message data and respond accordingly. This message is sent by the \"Error Handler\" VIs at the end of each loop in this application."
            n111 = property class="Mod Admin"(reference=w334) -> ("Accessors:External Launch"=w331:bool, "Accessors:Module ID"=w333:i32)  [unwired: 1 in, 2 out]
            n112 = Variant To Data(error in=w339, type=errorcluster {"status"=FALSE, "code"=0, "source"=""} ("error constant"), Variant=w337) -> (data=w340:errorcluster, error out=w335:errorcluster)
            n113 = call "Error Reported.vi"("Error"=w340, "Module ID"=w333) -> ()  [unwired: 9 in, 1 out]
            n114 = case shown="假" w331 {
              tunnel: [w345 _] -> w332
              tunnel: w330 -> [w344 _]
              tunnel: w340 -> [w341 _]
              frame False {
                # "If the module is running standalone, then pop up an error dialog and call the \"Exit\" message."
                n115 = call <vilib>:"Simple Error Handler.vi"("error in (no error)"=w341) -> ()  [unwired: 4 in, 5 out]
                n116 = call-poly <vilib>:"Delacor_lib_QMH_Enqueue Message (poly).vi"("Priority Message? (F)"=TRUE, "Message"="Exit", "Message Queue in"=w344) -> ("error out"=w345:errorcluster)  [unwired: 7 in, 1 out]
              }
              frame True {
                # "If the module was launched externally, calling the Error Reported broadcast VI is the only action performed by the \"Error\" message. The module's caller can then process the error appropriately."
              }
            }
            n117 = Merge Errors(w335, w332) -> (w329:errorcluster)
            n118 = local write "error out"(w329) -> ()
          }
          frame "Simulate MHL Error" {
            # "Simulate an error occurring at the MHL"
            n119 = property class="Mod Admin"(reference=w347) -> ("Accessors:Module ID"=w348:i32)  [unwired: 1 in, 2 out]
            n120 = call "Module Name--constant.vi"("Module ID"=w348) -> ("Module Name"=w346:string)  [unwired: 10 in]
            n121 = xnode "Error Ring"("参数 0"=w346) -> ("错误输出"=w349:errorcluster)
            n122 = Merge Errors(w352, w349) -> (w350:errorcluster)
          }
          frame "Confirm Quit" {
            # "#CodeNeeded - If you want to provide an \"Are you sure\" dialog (or some other notification) before the application exits, place that code here. This message is typically sent from a Panel Close? event."
            # "Confirm Quit - Message that can confirm whether or not the user wants to exit this instance."
            n123 = call-poly <vilib>:"Delacor_lib_QMH_Enqueue Message (poly).vi"("Priority Message? (F)"=TRUE, "error in"=w362, "Message"="Exit", "Message Queue in"=w363) -> ("error out"=w365:errorcluster)  [unwired: 6 in, 1 out]
            n124 = Merge Errors(w365) -> (w361:errorcluster)
          }
          frame "Exit" {
            w373 = 91  # 91: not all Exit messages will have an argument
            w377 = TRUE  # Stop the VI
            # "Release the message queue reference"
            # "#CodeNeeded - Add any required cleanup code here"
            # "Exit - Exit the application."
            n125 = Variant To Data(error in=w381, type=T5 {"Origin"="", "Module ID"=-1, "Exit via Stop Module Req?"=FALSE, "Wait for Module to stop?"=FALSE} ("Stop Argument"), Variant=w371) -> (data=w368:T5, error out=w372:errorcluster)
            n126 = call <vilib>:"Clear Errors.vi"("error in (no error)"=w372, "specific error code to clear (0: all)"=w373) -> ("error out"=w380:errorcluster)  [unwired: 4 in, 1 out]
            n127 = call-dynamic "Delacor_lib_QMH_Release Message Queue.vi"("error in"=w380, "Message Queue"=w379) -> ("error out"=w376:errorcluster)  [unwired: 9 in]
            n128 = call "Handle Exit.vi"("Stop Argument"=w368, "Module Admin in"=w367) -> ("error out"=w374:errorcluster, "Wait for Stop?"=w369:bool)  [unwired: 8 in]
            n129 = Merge Errors(w374, w376) -> (w375:errorcluster)
          }
          frame Default {
            # "'Default' case only runs if there is a message that isn't defined in any of the other cases.  Output a programming error."
            n130 = property class="Mod Admin"(reference=w383) -> ("Accessors:Module ID"=w382:i32)  [unwired: 1 in, 2 out]
            n131 = call "Module Name--constant.vi"("Module ID"=w382) -> ("Module Name"=w384:string)  [unwired: 10 in]
            n132 = xnode "Error Ring"("参数 0"=w385, "参数 1"=w384) -> ("错误输出"=w386:errorcluster)
          }
        }
        n133 = call-dynamic "Delacor_lib_QMH_Error Handler - Message Handling Loop.vi"("error in"=w236, "Message Queue in"=w227) -> ("dup error in"=w226:errorcluster)  [unwired: 8 in, 1 out]
      }
    }
    frame Error {
      n134 = call "Synchronize Caller Events.vi"("Module Admin"=w399) -> ("Module Admin out"=w398:refnum<class "Delacor_lib_QMH_Cloneable Module Admin.lvclass">)  [unwired: 9 in, 1 out]
      n135 = property class="Mod Admin"(reference=w398) -> ("Accessors:Module ID"=w397:i32)  [unwired: 1 in, 2 out]
      n136 = call "Module Name--constant.vi"("Module ID"=w397) -> ("Module Name"=w402:string)  [unwired: 10 in]
      n137 = call "Remove.vi"("Module ID"=w397) -> ()  [unwired: 9 in, 2 out]
      n138 = Format Into String(format string="An error occurred during initialization. %s is no longer running.", w402) -> (resulting string=w400:string)  [unwired: 2 in, 1 out]
      n139 = call "Error Reported.vi"("Additional Information"=w400, "Error"=w403, "Module ID"=w397) -> ()  [unwired: 8 in, 1 out]
    }
  }
  n140 = Unbundle By Name(w3) -> ("本VI"=w2:refnum<vi>)
  n141 = Merge Errors(w28, w27) -> (w29:errorcluster)
  n142 = call "Close Module.vi"("error in (no error)"=w29, "Wait for stop?"=w18, "Module Admin in"=w20) -> ("error out"=w22:errorcluster, "External Launch"=w16:bool, "Module Admin out"=w19:refnum<class "Delacor_lib_QMH_Cloneable Module Admin.lvclass">)  [unwired: 6 in]
  n143 = Close Reference(reference=w2) -> (error out=w1:errorcluster)  [unwired: 1 in]
  n144 = Unregister For Events(event registration refnum=w26, error in=w22) -> (error out=w17:errorcluster)
  "error out" <- w17
  n145 = call <vilib>:"Clear Errors.vi"("error in (no error)"=w1) -> ()  [unwired: 5 in, 2 out]
  n146 = local write "Module Admin"(w19) -> ()
  n147 = case "External Launch?" shown="真" w16 {
    tunnel: w17 -> [_ w409]
    tunnel: w12 -> [_ w407]
    tunnel: w6 -> [_ w405]
    frame False {
    }
    frame True {
      n148 = call-dynamic <vilib>:"Close.vi"("Panel In"=w407) -> ("Error Out"=w408:errorcluster)  [unwired: 10 in]
      n149 = call <vilib>:"Close.vi"("error in (no error)"=w408, "Controller in"=w405) -> ("error out"=w406:errorcluster)  [unwired: 9 in]
      n150 = case shown="无错误" w409 {
        tunnel: w406 -> [_ _]
        frame No Error {
        }
        frame Error {
          n151 = invoke class="VI" method="FP.Open"("Activate"=TRUE ("Activate?")) -> ()  [unwired: 4 in, 5 out]
        }
      }
    }
  }
